vi "Parse State Queue++.vi"(0 "State Queue":string, 1 "Name (\"\" to Use UUID)":string, 2 "Response Arguments":string, 7 "Previous Error":errorcluster, 9 "Dequeue (1 ms)":i32=1, 11 "Response Timeout (-2 Use Global Settings)":i32=-2, 12 "Allowed Messages (Empty for All)":string[](array[string])) -> (3 "Name Used":string, 4 "Remaining States":string, 6 "Current State":string, 8 "Arguments":string, 10 "Additional Information":T1, 15 "Source CSM":string)   [LabVIEW 2017, in "Communicable State Machine.lvlib"]
doc: "Parses the CSM state queue and returns the next current state to execute, along with arguments and other information.\n\n\n> [!NOTE] <b>CSM Inter-module Communication Types</b>\n>\n> Communication between CSM modules is divided into two categories: Messages and Broadcasts.\n> - <b>Messages</b>: 1:1 communication between modules. Based on the message handling method, it can be further divided into Synchronous Call (`-@`), Asynchronous Call (`->`), and Asynchronous Call without Reply (`->|`).\n> - <b>Broadcasts</b>: 1:N communication between modules. The broadcasting module pushes the broadcast to all modules registered to that broadcast. Based on the broadcast processing priority, it can be further divided into Status Broadcast and Interrupt Broadcast.\n\n\n-- <b>Controls</b> --\n- <b>Response Arguments</b>: Response arguments from the previous state. Connect this input to the CSM shift register to pass return values from external calls.\n- <b>Name (\"\" to use UUID)</b>: CSM module name. Refer to <b>CSM Naming Rules</b> for module naming rules.\n- <b>State Queue</b>: The entire state queue is connected to this input. This must be wired from a CSM shift register.\n- <b>Previous Error</b>: Error cluster from the CSM. If an error occurs and is passed to this input, the <b>Current State</b> output returns the `Error Handler` state.\n- <b>Dequeue (1 ms)</b>: Timeout setting for checking the CSM message queue. The default is 1 ms. The default is not set to 0 to avoid generating massive amounts of empty messages in certain error situations.\n- <b>Response Timeout (-2 Use Global Settings)</b>: Timeout for synchronous calls. The default is -2, which uses the global setting. You can set the global timeout using the CSM - Set TMO of Sync-Reply VI.\n- <b>Allowed Messages (Empty for All)</b>: A list of allowed message names. An empty list indicates that all messages are allowed.\n\n-- <b>Indicators</b> --\n- <b>Name Used</b>: Actual name assigned to the CSM module.\n- <b>Remaining States</b>: All concatenated states and arguments.\n- <b>Current State</b>: The next current state to execute.\n- <b>Arguments</b>: Returns any arguments that might be used in the current state string. These arguments are located after the `>>` characters.\n - Argument variables must not contain any non-printable characters, such as line feeds or carriage returns.\n- <b>Additional Information</b>: Supplemental information. For states triggered by a broadcast, this information contains the name and arguments of the broadcast.\n- <b>Source CSM</b>: If <b>Current State</b> is sent externally, this is the name of the source CSM module."
uses:
  Communicable State Machine.lvlib
  _Support/Typedef/_CSM_Response Source Message.ctl
  _Support/Typedef/_CSM_MSG_TYPE.ctl
  AdvanceAPI/CSM - Message Type.ctl
  _Support/FGV-BroadcastRegistry/Operation-BroadcastRegistry.ctl
  _Support/Typedef/_CSM_GlobalLog_MSG.ctl
  _Support/Typedef/_CSM_GlobalLog_MSG_TYPE.ctl
  _Support/Typedef/_CSM Status Change Event Data.ctl
  _Support/CSMQ/_CSMObj-Message Check.vi
  _Support/CSMQ/_CSMObj-Enqueue Cross-Module Message.vi
  _Support/CSMQ/_CSMOFGV Get.vi
  _Support/GlobalEvent/GEvt-Generate with Rule Check.vi
  AdvanceAPI/CSM - Make String Arguments Safe.vi
  _Support/Common/Hex Str to U8 Data.vi
  AdvanceAPI/CSM - Revert Arguments-Safe String.vi
  _Support/Common/U8 Data to Hex Str.vi
  _Support/Priority Queue/Dequeue Element.vi
  _Support/GlobalEvent/GEvt-Convert Filter Rules - v1.0.vi
  _Support/ChangeFlag/FlagInstance-GEvt Filter.vi
  _Support/ChangeFlag/FlagInstance-GEvt Refs.vi
  _Shared/CSM - System States.vi
  _Support/Priority Queue/Enqueue Element.vi
  AdvanceAPI/CSM - Keywords.vi
  _Support/ChangeFlag/ChangeFlag-Read.vi
  _Support/GlobalEvent/LogFilter/LogFilter - Check.vi
  AdvanceAPI/CSM - Module Status.vi
  AdvanceAPI/CSM - Resolve Node Module.vi
  _Support/CSMQ/_CSMOFGV(lvlibp).vi
  _Shared/Trim Single-line Text.vi
  _Polymophic/Build Synchronous Message with Arguments.vi
  _Support/CSMKVMap/CSMKVMap-Read.vi
  _Support/Error/CSM Not Allowed Message.vi
  _Support/FGV-BroadcastRegistry/FGV-BroadcastRegistry(lvlibp).vi
  _Support/CSMQ/_CSMObj-Add Internal Registry Rule.vi
  _Support/Message/Parse Unregister Message.vi
  _Support/Message/Parse Register Message.vi
  _Shared/Concatenate State with Arguments.vi
  _Support/Error/CSM Missing Return State Error.vi
  Utility/Build Internal State String.vi
  _Shared/Concatenate PostPostMsg Message.vi
  Utility/_openG/1D Array to String_csm.vi
  _Support/GlobalEvent/LogFilter/SettingVIs/Set CSM StateType Filter.vi
  _Support/GlobalEvent/LogFilter/SettingVIs/Set Global StateType Filter.vi
  _Support/GlobalEvent/LogFilter/SettingVIs/Set CSM State Filter.vi
  _Support/GlobalEvent/LogFilter/SettingVIs/Set CSM LogType Filter.vi
  _Support/GlobalEvent/LogFilter/SettingVIs/Set Global State Filter.vi
  _Support/GlobalEvent/LogFilter/SettingVIs/Set Global LogType Filter.vi
  _Support/GlobalEvent/LogFilter/SettingVIs/Set Global CSM Filter.vi
  _Support/GlobalEvent/FGV-GEvt Filter Rules(lvlibp).vi
  _Support/ChangeFlag/ChangeFlagDB.vi
  _Support/GlobalEvent/GEvt-Valid Subscribers.vi
  _Support/GlobalEvent/FGV-GlobalEventQueues(lvlibp).vi
  _Support/GlobalEvent/FGV-GlobalEventRef(lvlibp).vi
  _Support/GlobalEvent/LogFilter/LogFilter.lvclass
  _Shared/CSM Shared.lvlib
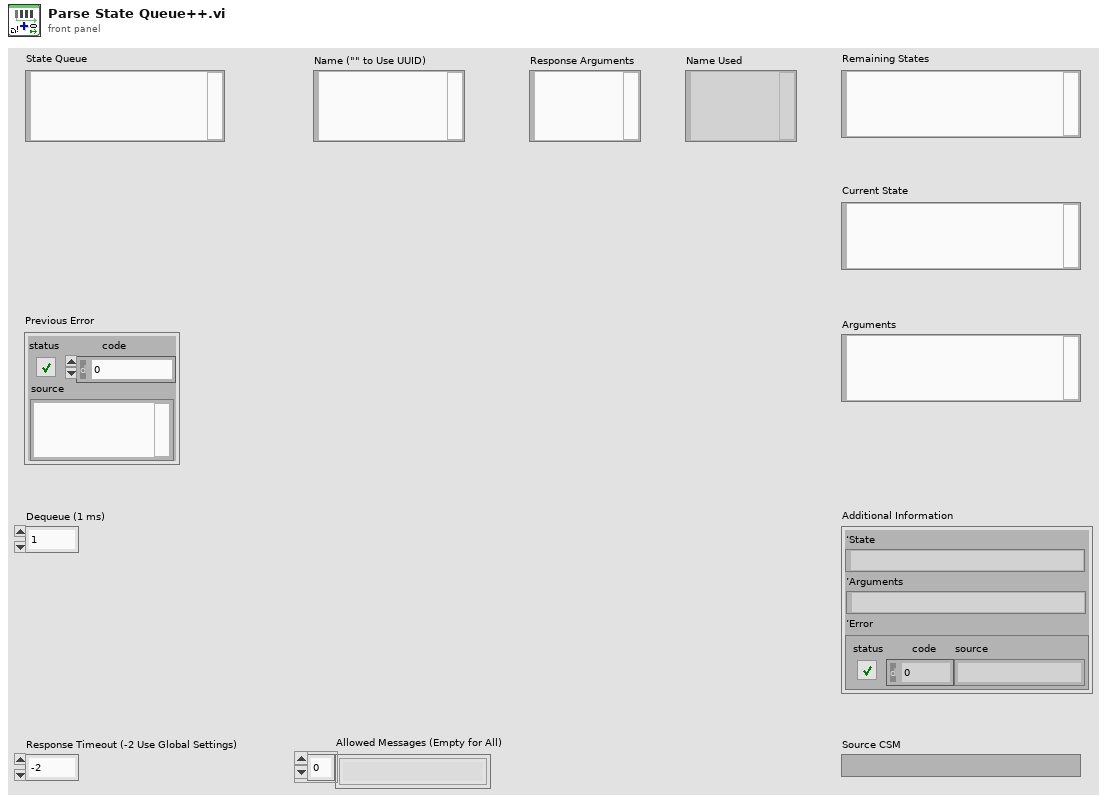
[diagram p1: front panel]
types:
  T1 = typedef "Communicable State Machine.lvlib/_CSM_Response Source Message.ctl" = cluster{"‘State":string, "’Arguments":string, "’Error":errorcluster}
  T2 = typedef "Communicable State Machine.lvlib/GEvt-Refs.ctl" = cluster{"Event":refnum<user-event>, "Queues":refnum<queue>[], "Valid":bool}
  T3 = typedef "Communicable State Machine.lvlib/_CSMObj.ctl" = cluster{"info":T4, "Refs":T6}
  T4 = typedef "Communicable State Machine.lvlib/_CSMObj-Info.ctl" = cluster{"Module Name":string, "Requested Name":string, "Group Name":string, "Mode":T5, "Allowed Messages":string[]}
  T5 = typedef "Communicable State Machine.lvlib/_CSM_MODE.ctl" = enum16{"Not Exist", "Stand Alone", "CSM", "Worker", "Worker Agent", "Chain Node", "Chain"}
  T6 = typedef "Communicable State Machine.lvlib/_CSMObj-Refs.ctl" = cluster{"WatchDogQ":refnum<queue>, "CSMDataDVR":refnum<data-value>, "Queue":T7, "GroupDataDVR":refnum<data-value>, "TagMap":refnum<data-value>, "ExitEvent":refnum<user-event>, "NewStateEvent":refnum<user-event>, "StatusEvent":refnum<user-event>, "InterruptEvent":refnum<user-event>}
  T7 = typedef "Communicable State Machine.lvlib/Priority Queue.ctl" = cluster{"HPriorityQ":refnum<queue>, "LowPriorityQ":refnum<queue>}
  T8 = typedef "Communicable State Machine.lvlib/CSM - Message Type.ctl" = enum16{"Async", "Async without Reply", "Sync"}
  T9 = typedef "Communicable State Machine.lvlib/_CSM_MSG_TYPE.ctl" = enum16{"Sync Message(-@)", "Async Message(->)", "Async without Response(->|)", "Async Response", "Broadcast(-><all>)", "Broadcast(-><status>)", "Broadcast(-><interrupt>)", "Append to JKISM States", "Append to JKISM States(High Priority)", "Broadcast(-><state>)", "<None>"}
  T10 = typedef "Communicable State Machine.lvlib/Operation-BroadcastRegistry.ctl" = enum16{"Delete Source Module", "Delete Target Module", "Remove Module", "Register", "Unregister", "Check", "List Status", "List Entries", "List Status Of Source", "Drop", "Register As Status", "Register As Interrupt"}
  T11 = typedef "Communicable State Machine.lvlib/_CSM_GlobalLog_MSG_TYPE.ctl" = enum16{"User Log", "State Change", "Status", "Interrupt", "Register", "Unregister", "Error Log", "Module Created", "Module Destroyed", "Async Message", "No-Rep Async Message", "Sync Message"}
  T12 = typedef "Communicable State Machine.lvlib/_CSM_GlobalLog_MSG.ctl" = cluster{"Name (\"\" to Use UUID)":string, "Current State":string, "Arguments":string, "Source Message":T1, "Source Module":string, "Complete(T)/Start(F)":bool, "LogType":T11, "Time Stamp":timestamp}
  T13 = typedef "Communicable State Machine.lvlib/_CSM Status Change Event Data.ctl" = cluster{"ModuleName":string, "Status":string, "Arguments":string}
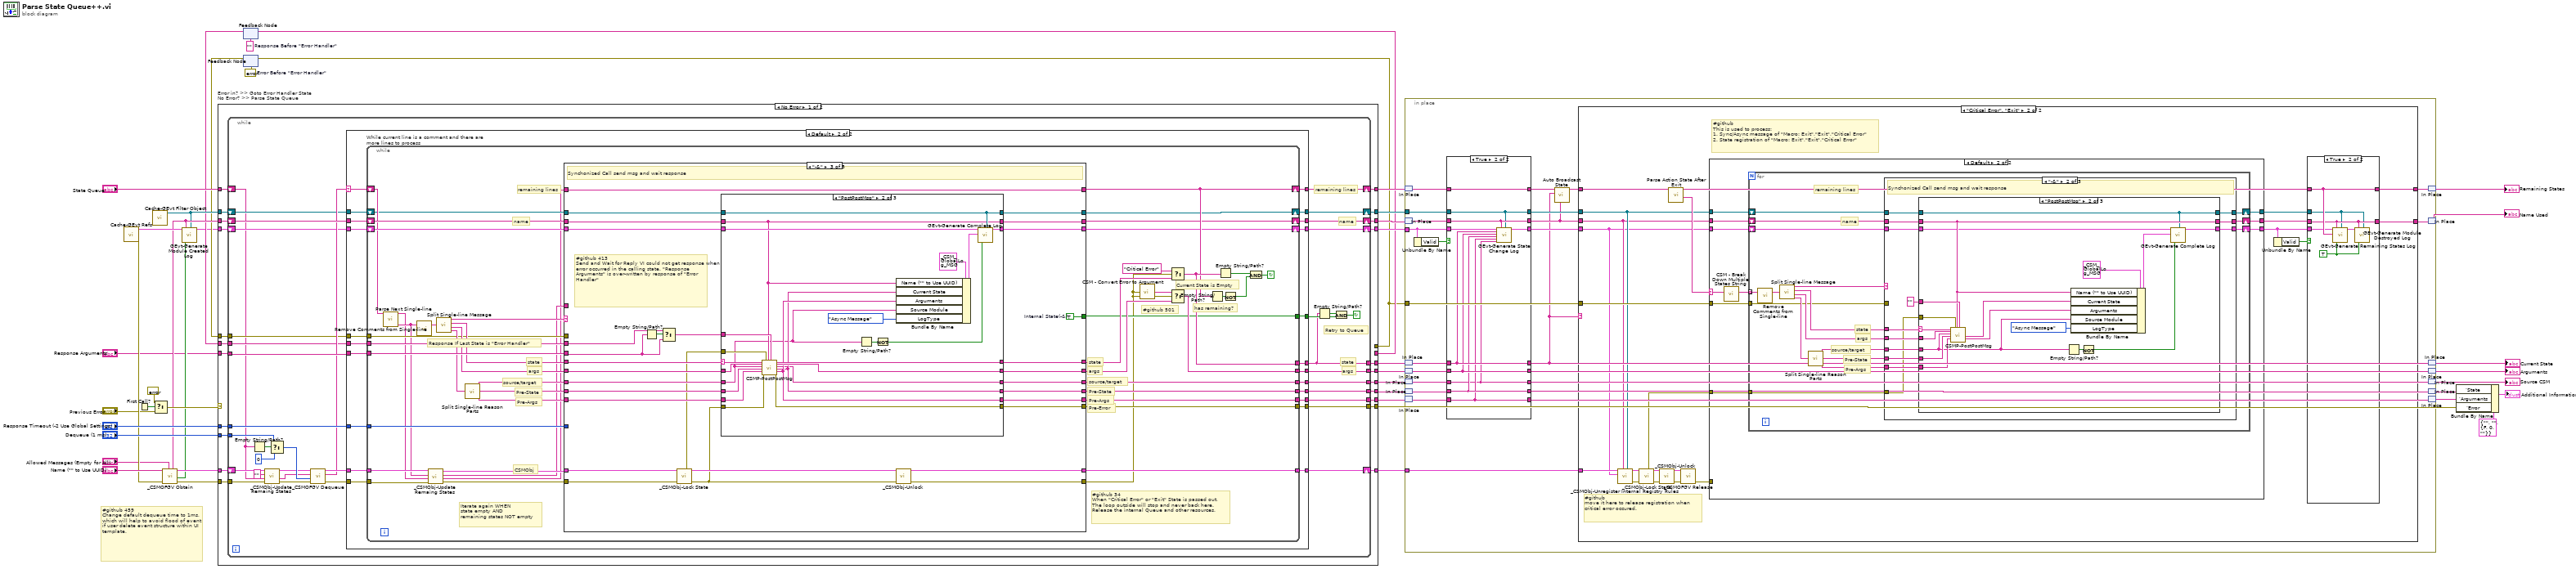
[diagram p0: block diagram]
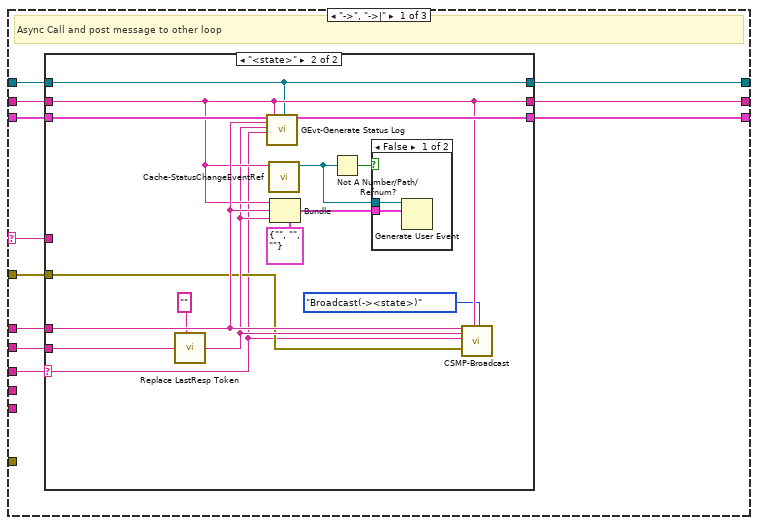
[diagram p4: hidden frame]
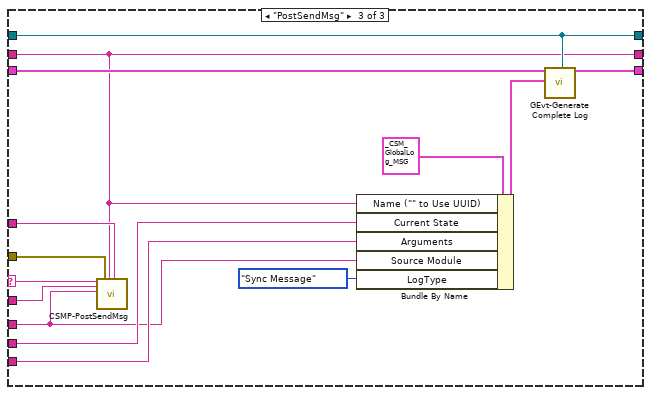
[diagram p8: hidden frame]
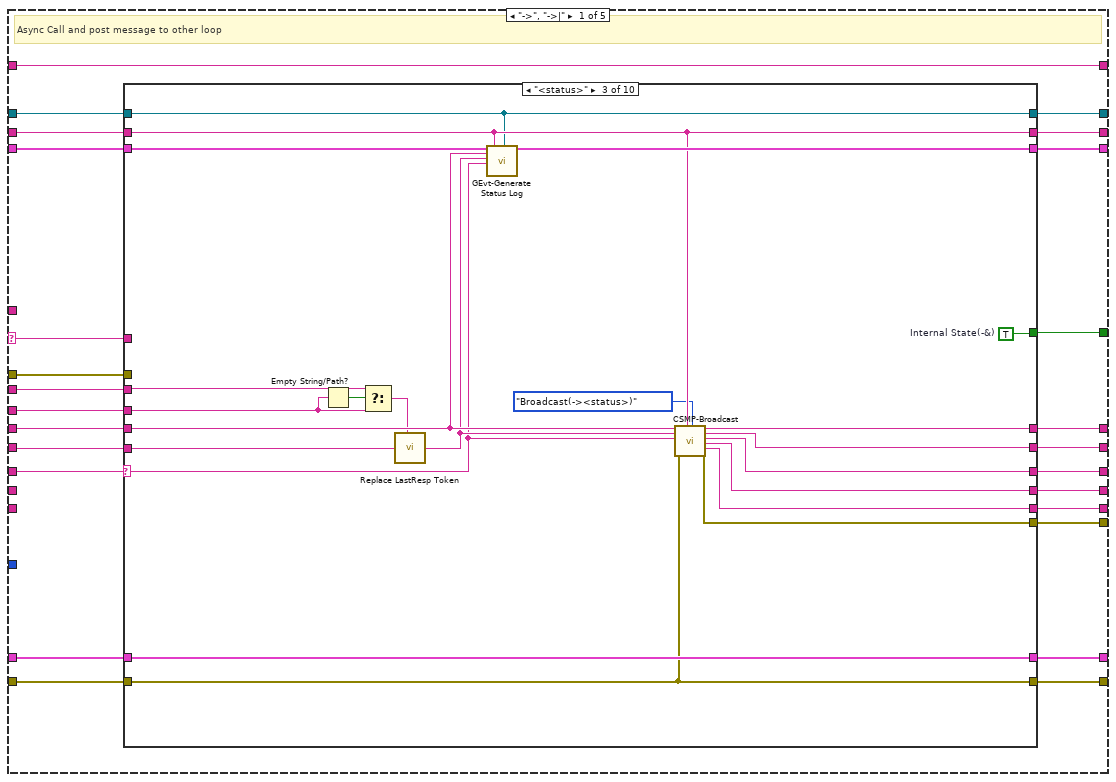
[diagram p13: hidden frame]
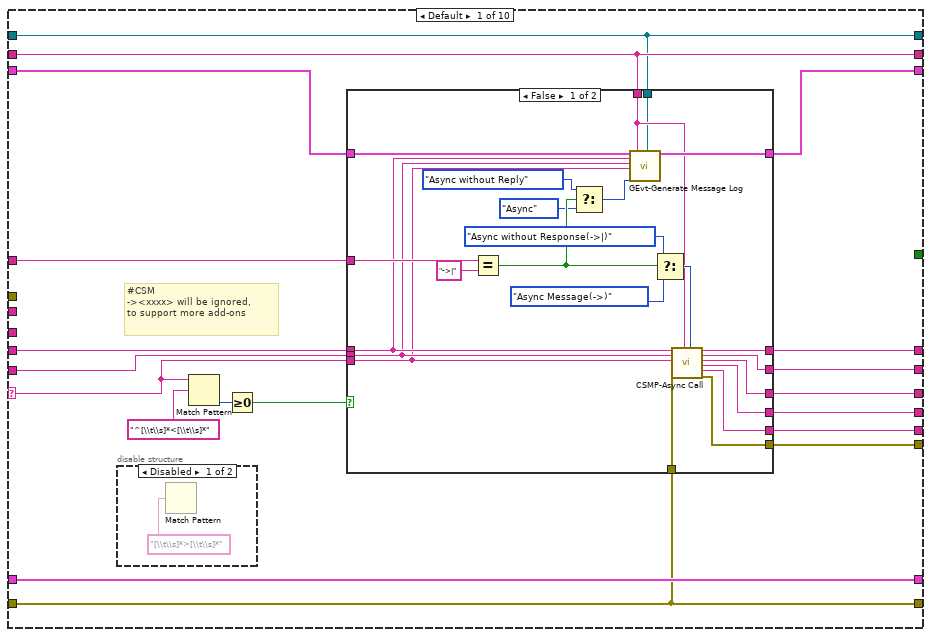
[diagram p14: hidden frame]
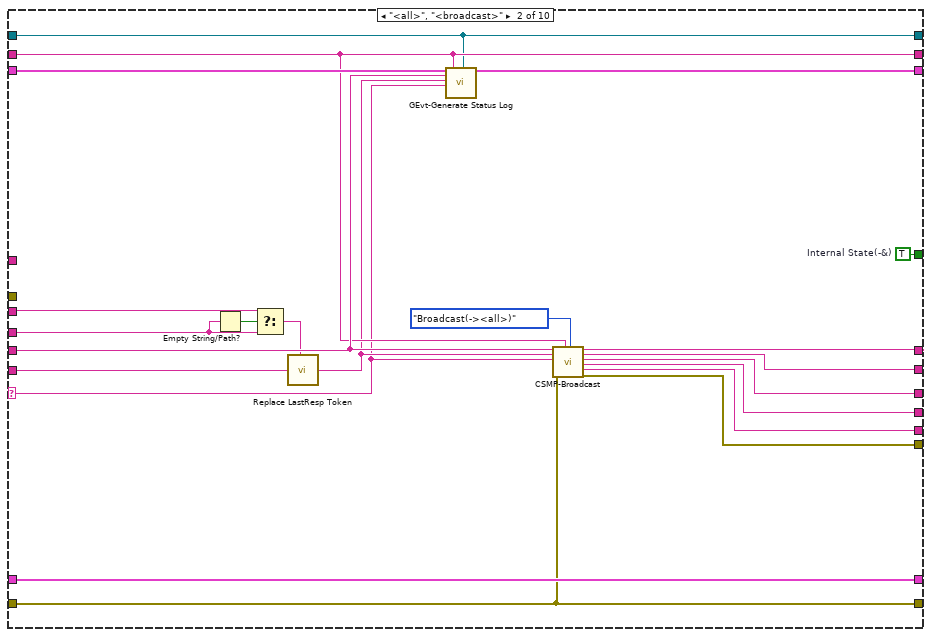
[diagram p17: hidden frame]
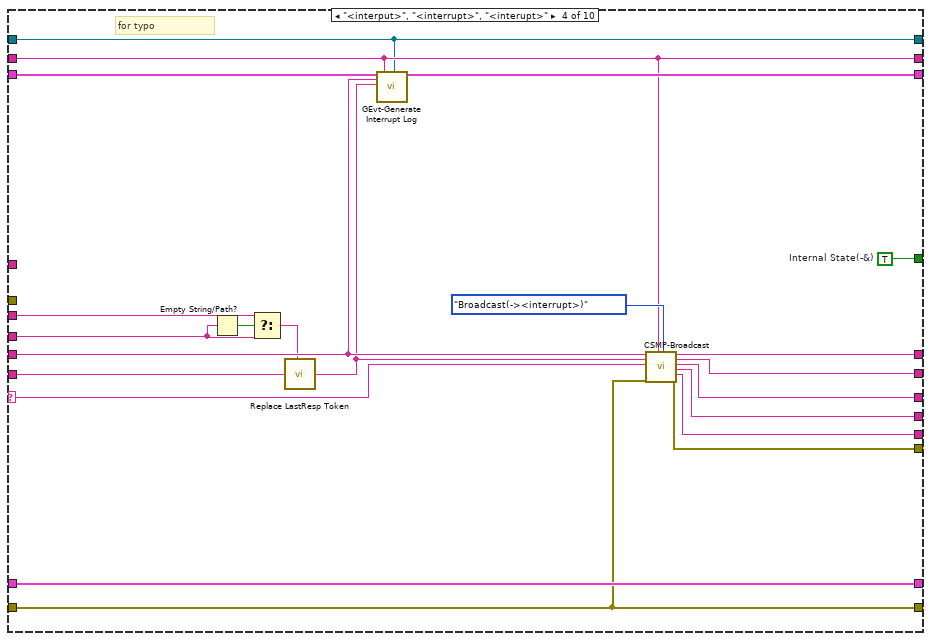
[diagram p18: hidden frame]
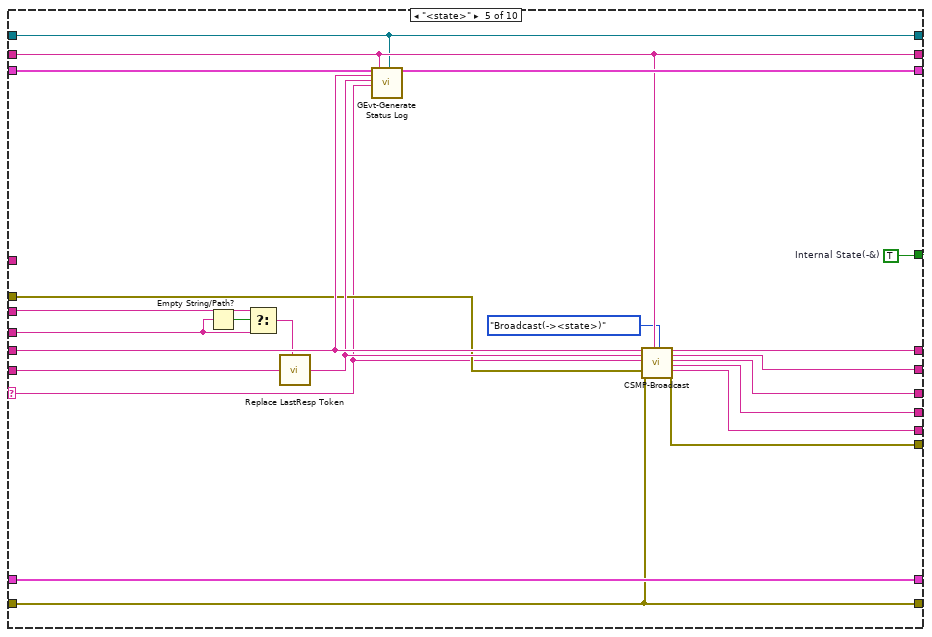
[diagram p19: hidden frame]
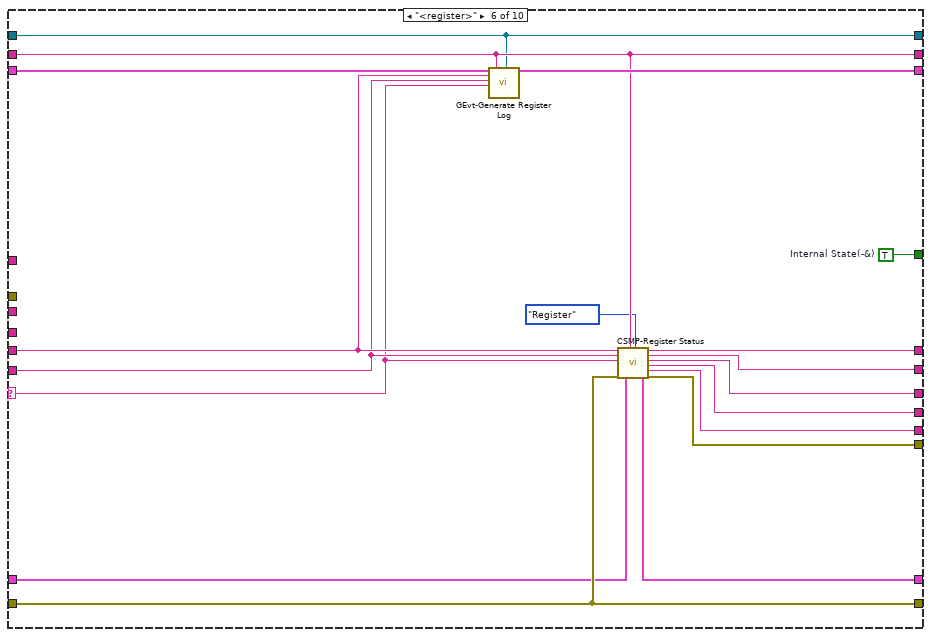
[diagram p20: hidden frame]
diagram:
  w5 = errorcluster {"status"=FALSE, "code"=0, "source"=""}  # Error Before "Error Handler"
  w8 = ""  # Response Before "Error Handler"
  # "#github 459\nChange default dequeue time to 1ms, which will help to avoid flood of event\nif user delete event structure within UI template."
  n1 = call "Cache-GEvt Refs.vi"() -> ("error out"=w28:errorcluster, "CSM Global Log Ref"=w14:T2)  [unwired: 10 in]
  n2 = First Call?() -> (First Call?: T/F=w18:bool)
  n3 = call "Cache-GEvt Filter Object.vi"() -> ("CSM:LogFilter.lvclass"=w10:refnum<class "LogFilter.lvclass">)  [unwired: 11 in]
  n4 = Select(t=errorcluster {"status"=FALSE, "code"=0, "source"=""}, s=w18, f="Previous Error") -> (s? t:f=w16:errorcluster)
  n5 = call "_CSMOFGV Obtain.vi"("Allowed Messages (Empty For All)"="Allowed Messages (Empty for All)", "Error In"=w28, "Name (\"\" to Use UUID) In"="Name (\"\" to Use UUID)") -> ("error out"=w41:errorcluster, "Create? (T)/Cached(F)"=w12:bool, "CSM-Obj"=w40:T3, "Name"=w13:string)  [unwired: 5 in]
  n6 = call "GEvt-Generate Module Created Log.vi"("CSM Global Log Event"=w14, "Name (\"\" to Use UUID)"=w13, "Created?"=w12, "CSM:LogFilter.lvclass"=w10) -> ("CSM Global Log Event Out"=w1:T2)  [unwired: 14 in, 1 out]
  n7 = feedback #1(w8) -> (w6:string)
  n8 = feedback #2(w5) -> (w4:errorcluster)
  n9 = case "Error in? >> Goto Error Handler State\nNo Error? >> Parse State Queue" shown="No Error" w16 {
    selector: w16 -> [_ w630]
    tunnel: [w64 w639] -> w31
    tunnel: [w66 "Error Handler"] -> w39
    tunnel: [w65 w635] -> w38
    tunnel: "State Queue" -> [w61 w639]
    tunnel: "Response Timeout (-2 Use Global Settings)" -> [w63 _]
    tunnel: w40 -> [w56 w634]
    tunnel: [w62 _] -> w36
    tunnel: "Dequeue (1 ms)" -> [w60 _]
    tunnel: [w59 _] -> w37
    tunnel: "Response Arguments" -> [w58 w631]
    tunnel: w41 -> [w57 w633]
    tunnel: w13 -> [w55 w637]
    tunnel: w1 -> [w54 w636]
    tunnel: [w53 w637] -> w27
    tunnel: [w52 w636] -> w26
    tunnel: [w51 _] -> w23
    tunnel: [w50 _] -> w20
    tunnel: w10 -> [w49 w632]
    tunnel: [w48 w632] -> w11
    tunnel: [_ w631] -> w7
    tunnel: w6 -> [w47 _]
    tunnel: [_ w630] -> w3
    tunnel: w4 -> [w46 _]
    tunnel: [w45 w629] -> w2
    frame No Error {
      n10 = while {
        tunnel: [w101] -> w65
        tunnel: w63 -> [w99]
        tunnel: [w98] -> w62
        tunnel: w60 -> [w95]
        tunnel: w57 -> [w73]
        shift-right: [w100] -> w64
        shift-left: w61 -> [w69]
        tunnel: w58 -> [w91]
        tunnel: [w85] -> w66
        tunnel: [w92] -> w59
        shift-right: [w82] -> w53
        shift-left: w55 -> [w90]
        shift-right: [w81] -> w52
        shift-left: w54 -> [w83]
        tunnel: [w80] -> w51
        tunnel: [w79] -> w50
        shift-right: [w77] -> w48
        shift-left: w49 -> [w78]
        tunnel: w47 -> [w76]
        tunnel: w46 -> [w75]
        shift-right: [w74] -> w45
        shift-left: w56 -> [w72]
        stop <- w87 continue-if-true
        # "args"
        # "state"
        # "name"
        # "remaining lines"
        # "Retry to Queue"
        n11 = Empty String/Path?(string/path=w69) -> (empty?=w96:bool)
        n12 = call "_CSMObj-Update Remaing States.vi"("Error In"=w73, "Remaing JKISM Queue"=w69, "Current State"="", "CSMQ In"=w72) -> ("error out"=w70:errorcluster, "Remaing JKISM Queue(dup)"=w68:string, "CSMQ Out"=w71:T3)  [unwired: 4 in, 1 out]
        n13 = Select(t=w95, s=w96, f=0) -> (s? t:f=w93:i32)
        n14 = call "_CSMOFGV Dequeue.vi"("Error In"=w70, "Dequeue Timeout (0ms)"=w93, "State (S) In (\"\")"=w68, "CSMQ In"=w71) -> ("error out"=w88:errorcluster, "States Out"=w89:string, "CSMQ Out"=w97:T3)  [unwired: 5 in]
        n15 = case shown="Default" w89 {
          selector: w89 -> [_ w121]
          tunnel: [_ w127] -> w85
          tunnel: [_ w126] -> w101
          tunnel: [_ w125] -> w100
          tunnel: w99 -> [_ w124]
          tunnel: [_ w123] -> w98
          tunnel: w90 -> [w105 w122]
          tunnel: w97 -> [w102 w120]
          tunnel: w88 -> [_ w119]
          tunnel: [_ w118] -> w92
          tunnel: w91 -> [_ w117]
          tunnel: [_ w116] -> w86
          tunnel: w83 -> [w104 w115]
          tunnel: [w105 w114] -> w82
          tunnel: [w104 w113] -> w81
          tunnel: [_ w112] -> w80
          tunnel: [_ w111] -> w79
          tunnel: w78 -> [w103 w110]
          tunnel: [w103 w109] -> w77
          tunnel: w76 -> [_ w108]
          tunnel: w75 -> [_ w107]
          tunnel: [w102 w106] -> w74
          frame "" {
            # "Dispatch Mode\n1. Error will Occurred\n2. Add Macro: Exit\n3. The Queue will regenerated\n4. But it will go Through Macro: Exit\n5. After Exit(queue released), then another Worker will be triggered."
            # "Do Nothing if Empty String"
            # "<< Wiring into the Case Selector is much more performant than using \"Empty String/Path?\" primitive"
          }
          frame Default {
            n16 = while "While current line is a comment and there are more lines to process" {
              tunnel: [w162] -> w127
              tunnel: [w164] -> w126
              shift-right: [w158] -> w125
              shift-left: w121 -> [w150]
              tunnel: w124 -> [w169]
              tunnel: [w163] -> w123
              tunnel: w120 -> [w134]
              tunnel: w119 -> [w135]
              tunnel: [w168] -> w118
              tunnel: w117 -> [w167]
              tunnel: [w160] -> w116
              shift-right: [w141] -> w114
              shift-left: w122 -> [w157]
              shift-right: [w139] -> w113
              shift-left: w115 -> [w156]
              tunnel: [w155] -> w112
              tunnel: [w145] -> w111
              shift-right: [w140] -> w109
              shift-left: w110 -> [w142]
              tunnel: w108 -> [w144]
              tunnel: w107 -> [w143]
              tunnel: [w138] -> w106
              stop <- w159 continue-if-true
              # "#github 501"
              # "Response If Last State is \"Error Handler\""
              # "source/target"
              # "Pre-Error"
              # "args"
              # "state"
              # "Pre-Args"
              # "Pre-State"
              # "source/target"
              # "Pre-Args"
              # "Pre-State"
              # "CSMObj"
              # "#github 34\nWhen \"Critical Error\" or \"Exit\" State is passed out,\nThe loop outside will stop and never back here.\nRelease the internal Queue and other resources."
              # "name"
              # "remaining lines"
              # "Iterate again WHEN\nstate empty AND\nremaining states NOT empty"
              # "args"
              # "state"
              # "Current State is Empty"
              # "has remaining?"
              n17 = call "Parse Next Single-line.vi"("States Queue"=w150) -> ("Next Single-line State"=w131:string, "Remaining States Queue"=w130:string)  [unwired: 9 in]
              n18 = call "Remove Comments from Single-line.vi"("single-line text"=w131) -> ("single-line text without comments"=w154:string)  [unwired: 2 in]
              n19 = call "_CSMObj-Update Remaing States.vi"("Error In"=w135, "Remaing JKISM Queue"=w130, "Current State"=w131, "CSMQ In"=w134) -> ("error out"=w132:errorcluster, "Remaing JKISM Queue(dup)"=w128:string, "Current State(dup)"=w129:string, "CSMQ Out"=w133:T3)  [unwired: 4 in]
              n20 = call "Split Single-line Message.vi"("single-line text"=w154) -> ("operator"=w151:string, "state"=w152:string, "args"=w153:string, "source/target"=w149:string)  [unwired: 6 in]
              n21 = call "Split Single-line Reason Parts.vi"("Single-line -& Reason"=w149) -> ("CSM Name"=w148:string, "`State"=w147:string, "`Arguments"=w146:string)  [unwired: 12 in]
              n22 = case shown="\"-&\"" w151 {
                selector: w151 -> [w186 _ _ _ _]
                tunnel: w152 -> [w194 w423 w463 w537 w628]
                tunnel: w153 -> [w193 w422 w465 w536 w627]
                tunnel: [w197 w435 w467 w535 w628] -> w166
                tunnel: [w196 w434 w466 w534 w627] -> w165
                tunnel: w157 -> [w192 w425 w457 w529 w621]
                tunnel: w148 -> [w195 w421 w456 w532 w624]
                tunnel: w169 -> [_ w428 _ _ _]
                tunnel: w133 -> [w184 w437 w451 w543 w625]
                tunnel: w128 -> [w187 w436 w459 w539 w623]
                tunnel: [w191 w432 w462 w531 _] -> w168
                tunnel: w167 -> [w189 _ w445 _ _]
                tunnel: w132 -> [w190 w429 w450 w542 w626]
                tunnel: [w177 w429 w464 w541 w626] -> w137
                tunnel: [w179 w433 w453 w533 w624] -> w163
                tunnel: [w185 w437 w461 w540 w625] -> w138
                tunnel: [w188 _ w460 w527 _] -> w160
                tunnel: [w187 w436 w459 w538 w623] -> w158
                tunnel: w156 -> [w183 w427 w438 w528 w622]
                tunnel: [w182 w426 w439 w528 w622] -> w139
                tunnel: [w180 w431 w458 w522 _] -> w155
                tunnel: [w181 w425 w442 w529 w621] -> w141
                tunnel: w147 -> [_ _ w455 w530 _]
                tunnel: w146 -> [_ _ w454 w523 _]
                tunnel: [w178 w430 w452 w521 _] -> w145
                tunnel: w142 -> [w176 w424 w440 w520 w620]
                tunnel: w129 -> [_ _ _ w526 _]
                tunnel: w144 -> [w175 _ w444 _ _]
                tunnel: w143 -> [w174 _ _ _ _]
                tunnel: [w173 w424 w441 w520 w620] -> w140
                frame "->", "->|" {
                  # "Async Call and post message to other loop"
                  n23 = case shown="\"<status>\"" w195 {
                    selector: w195 -> [w203 w246 w268 w301 w312 w334 w352 w370 w402 _]
                    tunnel: [w211 w252 w281 w300 w328 w349 w367 w385 w401 _] -> w197
                    tunnel: [w210 w253 w278 w299 w325 w348 w366 w384 w400 _] -> w196
                    tunnel: w194 -> [w216 w262 w282 w303 w329 w338 w356 w374 w390 w406]
                    tunnel: w193 -> [w212 w261 w279 w302 w326 w337 w355 w373 w389 _]
                    tunnel: w192 -> [w213 w260 w280 w305 w327 w339 w357 w375 w391 w412]
                    tunnel: [w209 w255 w276 w297 w323 w346 w364 w382 w398 _] -> w191
                    tunnel: w190 -> [w205 w258 w284 w304 w314 w350 w368 w386 w403 w408]
                    tunnel: w189 -> [_ w248 w271 w291 w318 _ _ _ _ _]
                    tunnel: [_ w266 w288 w310 w333 w351 w369 w387 w404 TRUE ("Internal State(-&)")] -> w188
                    tunnel: w186 -> [w215 _ _ _ _ _ _ _ _ _]
                    tunnel: [w214 w265 w287 w309 w315 w342 w360 w378 w394 w410] -> w185
                    tunnel: w184 -> [w214 w265 w287 w309 w315 w343 w361 w379 w395 w409]
                    tunnel: [w199 w264 w285 w307 w331 w340 w358 w376 w392 w413] -> w182
                    tunnel: w183 -> [w200 w263 w286 w308 w332 w341 w359 w377 w393 w413]
                    tunnel: [w213 w260 w280 w305 w327 w339 w357 w375 w391 w412] -> w181
                    tunnel: [w208 w256 w275 w296 w322 w345 w363 w381 w397 _] -> w180
                    tunnel: [w207 w254 w277 w298 w324 w347 w365 w383 w399 _] -> w179
                    tunnel: [w206 w257 w283 w295 w330 w344 w362 w380 w396 _] -> w178
                    tunnel: [w205 w258 w284 w304 w314 w350 w368 w386 w403 w407] -> w177
                    tunnel: w176 -> [w198 w245 w267 w289 w311 w336 w354 w372 w388 w405]
                    tunnel: w175 -> [_ w249 w270 w292 w317 _ _ _ _ _]
                    tunnel: w174 -> [_ _ _ _ w313 _ _ _ _ _]
                    tunnel: [w198 w245 w267 w289 w311 w336 w354 w372 w388 w405] -> w173
                    frame Default {
                      # "#CSM\n-><xxxx> will be ignored,\nto support more add-ons"
                      n24 = disable-structure shown="Disabled" {
                        frame Disabled {
                          n25 = Match Pattern(regular expression="[\\t\\s]*>[\\t\\s]*") -> ()  [unwired: 2 in, 4 out]
                        }
                        frame Enabled {
                        }
                      }
                      n26 = Match Pattern(string=w203, regular expression="^[\\t\\s]*<[\\t\\s]*") -> (offset past match=w202:i32)  [unwired: 1 in, 3 out]
                      n27 = Greater Or Equal To 0?(x=w202) -> (x >= 0?=w201:bool)
                      n28 = case shown="False" w201 {
                        tunnel: w216 -> [w224 w244]
                        tunnel: w215 -> [w240 _]
                        tunnel: w213 -> [w226 _]
                        tunnel: w212 -> [w223 w243]
                        tunnel: [w236 w244] -> w211
                        tunnel: [w235 w243] -> w210
                        tunnel: [w234 _] -> w209
                        tunnel: [w233 _] -> w208
                        tunnel: [w232 w242] -> w207
                        tunnel: [w231 _] -> w206
                        tunnel: w205 -> [w229 _]
                        tunnel: w203 -> [w222 w242]
                        tunnel: w200 -> [w228 w241]
                        tunnel: [w227 w241] -> w199
                        tunnel: w198 -> [w225 _]
                        frame False {
                          n29 = Equal?(x=w240, y="->|") -> (x = y?=w220:bool)
                          n30 = Select(t=CSM_-_Message_Type."Async without Reply" ("Type"), s=w220, f=CSM_-_Message_Type."Async" ("Type")) -> (s? t:f=w218:T8)
                          n31 = call "GEvt-Generate Message Log.vi"("CSM Global Log Event"=w228, "Current State"=w224, "Arguments"=w223, "Source Module"=w222, "Type"=w218, "Name (\"\" to Use UUID)"=w226, "CSM:LogFilter.lvclass"=w225) -> ("CSM Global Log Event Out"=w227:T2)  [unwired: 11 in, 1 out]
                          n32 = Select(t=_CSM_MSG_TYPE."Async without Response(->|)" ("Msg Type"), s=w220, f=_CSM_MSG_TYPE."Async Message(->)" ("Msg Type")) -> (s? t:f=w230:T9)
                          n33 = call "CSMP-Async Call.vi"("State"=w224, "Args"=w223, "Source/target"=w222, "Error In"=w229, "Module Name"=w226, "Msg Type"=w230) -> ("State Out"=w236:string, "Args Out"=w235:string, "Source/target Out"=w232:string, "Pre-State Out"=w234:string, "Pre-Args Out"=w233:string, "Error"=w231:errorcluster)  [unwired: 8 in]
                        }
                        frame True {
                        }
                      }
                    }
                    frame "<all>", "<broadcast>" {
                      w266 = TRUE  # Internal State(-&)
                      n34 = Empty String/Path?(string/path=w248) -> (empty?=w250:bool)
                      n35 = Select(t=w249, s=w250, f=w248) -> (s? t:f=w247:string)
                      n36 = call "Replace LastResp Token.vi"("LastResp"=w247, "Argument"=w261) -> ("Argument Out"=w251:string)  [unwired: 5 in]
                      n37 = call "GEvt-Generate Status Log.vi"("CSM Global Log Event"=w263, "Current State"=w262, "Arguments"=w251, "Source Module"=w246, "Name (\"\" to Use UUID)"=w260, "CSM:LogFilter.lvclass"=w245) -> ("CSM Global Log Event Out"=w264:T2)  [unwired: 12 in, 1 out]
                      n38 = call "CSMP-Broadcast.vi"("State"=w262, "Args"=w251, "Source/target"=w246, "Error In"=w258, "Module Name"=w260, "Msg Type"=_CSM_MSG_TYPE."Broadcast(-><all>)") -> ("State Out"=w252:string, "Args Out"=w253:string, "Source/target Out"=w254:string, "Pre-State Out"=w255:string, "Pre-Args Out"=w256:string, "Error"=w257:errorcluster)  [unwired: 8 in]
                    }
                    frame "<status>" {
                      w288 = TRUE  # Internal State(-&)
                      n39 = Empty String/Path?(string/path=w271) -> (empty?=w272:bool)
                      n40 = Select(t=w270, s=w272, f=w271) -> (s? t:f=w269:string)
                      n41 = call "Replace LastResp Token.vi"("LastResp"=w269, "Argument"=w279) -> ("Argument Out"=w273:string)  [unwired: 5 in]
                      n42 = call "GEvt-Generate Status Log.vi"("CSM Global Log Event"=w286, "Current State"=w282, "Arguments"=w273, "Source Module"=w268, "Name (\"\" to Use UUID)"=w280, "CSM:LogFilter.lvclass"=w267) -> ("CSM Global Log Event Out"=w285:T2)  [unwired: 12 in, 1 out]
                      n43 = call "CSMP-Broadcast.vi"("State"=w282, "Args"=w273, "Source/target"=w268, "Error In"=w284, "Module Name"=w280, "Msg Type"=_CSM_MSG_TYPE."Broadcast(-><status>)") -> ("State Out"=w281:string, "Args Out"=w278:string, "Source/target Out"=w277:string, "Pre-State Out"=w276:string, "Pre-Args Out"=w275:string, "Error"=w283:errorcluster)  [unwired: 8 in]
                    }
                    frame "<interput>", "<interrupt>", "<interupt>" {
                      w310 = TRUE  # Internal State(-&)
                      # "for typo"
                      n44 = Empty String/Path?(string/path=w291) -> (empty?=w293:bool)
                      n45 = Select(t=w292, s=w293, f=w291) -> (s? t:f=w290:string)
                      n46 = call "Replace LastResp Token.vi"("LastResp"=w290, "Argument"=w302) -> ("Argument Out"=w294:string)  [unwired: 5 in]
                      n47 = call "GEvt-Generate Interrupt Log.vi"("CSM Global Log Event"=w308, "Current State"=w303, "Arguments"=w294, "Name (\"\" to Use UUID)"=w305, "CSM:LogFilter.lvclass"=w289) -> ("CSM Global Log Event Out"=w307:T2)  [unwired: 13 in, 1 out]
                      n48 = call "CSMP-Broadcast.vi"("State"=w303, "Args"=w294, "Source/target"=w301, "Error In"=w304, "Module Name"=w305, "Msg Type"=_CSM_MSG_TYPE."Broadcast(-><interrupt>)") -> ("State Out"=w300:string, "Args Out"=w299:string, "Source/target Out"=w298:string, "Pre-State Out"=w297:string, "Pre-Args Out"=w296:string, "Error"=w295:errorcluster)  [unwired: 8 in]
                    }
                    frame "<state>" {
                      w333 = TRUE  # Internal State(-&)
                      n49 = Empty String/Path?(string/path=w318) -> (empty?=w319:bool)
                      n50 = Select(t=w317, s=w319, f=w318) -> (s? t:f=w316:string)
                      n51 = call "Replace LastResp Token.vi"("LastResp"=w316, "Argument"=w326) -> ("Argument Out"=w320:string)  [unwired: 5 in]
                      n52 = call "GEvt-Generate Status Log.vi"("CSM Global Log Event"=w332, "Current State"=w329, "Arguments"=w320, "Source Module"=w312, "Name (\"\" to Use UUID)"=w327, "CSM:LogFilter.lvclass"=w311) -> ("CSM Global Log Event Out"=w331:T2)  [unwired: 12 in, 1 out]
                      n53 = call "CSMP-Broadcast.vi"("State"=w329, "Args"=w320, "Source/target"=w312, "Response For Message.’Error"=w313, "Error In"=w314, "Module Name"=w327, "Msg Type"=_CSM_MSG_TYPE."Broadcast(-><state>)") -> ("State Out"=w328:string, "Args Out"=w325:string, "Source/target Out"=w324:string, "Pre-State Out"=w323:string, "Pre-Args Out"=w322:string, "Error"=w330:errorcluster)  [unwired: 7 in]
                    }
                    frame "<register>" {
                      w351 = TRUE  # Internal State(-&)
                      n54 = call "GEvt-Generate Register Log.vi"("CSM Global Log Event"=w341, "Current State"=w338, "Arguments"=w337, "Source Module"=w334, "Name (\"\" to Use UUID)"=w339, "CSM:LogFilter.lvclass"=w336) -> ("CSM Global Log Event Out"=w340:T2)  [unwired: 12 in, 1 out]
                      n55 = call "CSMP-Register Status.vi"("State"=w338, "Args"=w337, "Source/target"=w334, "Error In"=w350, "CSMQ In"=w343, "Module Name"=w339, "Operation"=Operation-BroadcastRegistry."Register") -> ("CSMQ Out"=w342:T3, "State Out"=w349:string, "Args Out"=w348:string, "Source/target Out"=w347:string, "Pre-State Out"=w346:string, "Pre-Args Out"=w345:string, "Error"=w344:errorcluster)  [unwired: 6 in]
                    }
                    frame "<register as status>" {
                      w369 = TRUE  # Internal State(-&)
                      n56 = call "GEvt-Generate Register Log.vi"("CSM Global Log Event"=w359, "Current State"=w356, "Arguments"=w355, "Source Module"=w352, "Name (\"\" to Use UUID)"=w357, "CSM:LogFilter.lvclass"=w354) -> ("CSM Global Log Event Out"=w358:T2)  [unwired: 12 in, 1 out]
                      n57 = call "CSMP-Register Status.vi"("State"=w356, "Args"=w355, "Source/target"=w352, "Error In"=w368, "CSMQ In"=w361, "Module Name"=w357, "Operation"=Operation-BroadcastRegistry."Register As Status") -> ("CSMQ Out"=w360:T3, "State Out"=w367:string, "Args Out"=w366:string, "Source/target Out"=w365:string, "Pre-State Out"=w364:string, "Pre-Args Out"=w363:string, "Error"=w362:errorcluster)  [unwired: 6 in]
                    }
                    frame "<register as interput>", "<register as interrupt>", "<register as interupt>" {
                      w387 = TRUE  # Internal State(-&)
                      n58 = call "GEvt-Generate Register Log.vi"("CSM Global Log Event"=w377, "Current State"=w374, "Arguments"=w373, "Source Module"=w370, "Name (\"\" to Use UUID)"=w375, "CSM:LogFilter.lvclass"=w372) -> ("CSM Global Log Event Out"=w376:T2)  [unwired: 12 in, 1 out]
                      n59 = call "CSMP-Register Status.vi"("State"=w374, "Args"=w373, "Source/target"=w370, "Error In"=w386, "CSMQ In"=w379, "Module Name"=w375, "Operation"=Operation-BroadcastRegistry."Register As Interrupt") -> ("CSMQ Out"=w378:T3, "State Out"=w385:string, "Args Out"=w384:string, "Source/target Out"=w383:string, "Pre-State Out"=w382:string, "Pre-Args Out"=w381:string, "Error"=w380:errorcluster)  [unwired: 6 in]
                    }
                    frame "<unregister>" {
                      w404 = TRUE  # Internal State(-&)
                      n60 = call "GEvt-Generate Unregister Log.vi"("CSM Global Log Event"=w393, "Current State"=w390, "Arguments"=w389, "Name (\"\" to Use UUID)"=w391, "CSM:LogFilter.lvclass"=w388) -> ("CSM Global Log Event Out"=w392:T2)  [unwired: 13 in, 1 out]
                      n61 = call "CSMP-Unregister Status.vi"("State"=w390, "Args"=w389, "Source/target"=w402, "Error In"=w403, "CSMQ In"=w395, "Module Name"=w391) -> ("CSMQ Out"=w394:T3, "State Out"=w401:string, "Args Out"=w400:string, "Source/target Out"=w399:string, "Pre-State Out"=w398:string, "Pre-Args Out"=w397:string, "Error"=w396:errorcluster)  [unwired: 7 in]
                    }
                    frame "<complete>" {
                      n62 = case shown="\"Macro: Initialize\"" w406 {
                        tunnel: [w415 w416] -> w410
                        tunnel: w409 -> [w415 w417]
                        tunnel: w408 -> [w414 w419]
                        tunnel: [w414 w418] -> w407
                        frame Default {
                        }
                        frame "Macro: Initialize" {
                          n63 = call "_CSMObj-Mark as Initialized.vi"("Error In"=w419, "CSMQ In"=w417) -> ("error out"=w418:errorcluster, "CSMQ Out"=w416:T3)  [unwired: 8 in]
                        }
                      }
                    }
                  }
                }
                frame "-@" {
                  # "Synchonized Call send msg and wait response"
                  n64 = call "GEvt-Generate Message Log.vi"("CSM Global Log Event"=w427, "Current State"=w423, "Arguments"=w422, "Source Module"=w421, "Type"=CSM_-_Message_Type."Sync", "Name (\"\" to Use UUID)"=w425, "CSM:LogFilter.lvclass"=w424) -> ("CSM Global Log Event Out"=w426:T2)  [unwired: 11 in, 1 out]
                  n65 = call "CSMP-Sync Call.vi"("State"=w423, "Args"=w422, "Source/target"=w421, "Error In"=w429, "Response Timeout (-2 Using Global Settings)"=w428, "Module Name"=w425) -> ("State Out"=w435:string, "Args Out"=w434:string, "Source/target Out"=w433:string, "Pre-State Out"=w432:string, "Pre-Args Out"=w431:string, "Error"=w430:errorcluster)  [unwired: 8 in]
                }
                frame "-&" {
                  w460 = TRUE  # Internal State(-&)
                  # "#github 413\nSend and Wait for Reply VI could not get response when error occurred in the calling state. \"Response Arguments\" is over-written by response of \"Error Handler\""
                  # "Synchonized Call send msg and wait response"
                  n66 = Empty String/Path?(string/path=w445) -> (empty?=w446:bool)
                  n67 = Select(t=w444, s=w446, f=w445) -> (s? t:f=w443:string)
                  n68 = call "_CSMObj-Lock State.vi"("Error In"=w450, "CSMQ In"=w451) -> ("error out"=w448:errorcluster, "CSMQ Out"=w449:T3, "Error"=w447:errorcluster)  [unwired: 5 in, 1 out]
                  n69 = case shown="\"PostPostMsg\"" w463 {
                    selector: w463 -> [w473 w497 w519]
                    tunnel: ["Critical Error" ("before match") w492 w518] -> w467
                    tunnel: [w475 w493 w516] -> w466
                    tunnel: w456 -> [_ w478 w501]
                    tunnel: w465 -> [_ w496 w517]
                    tunnel: w443 -> [_ w498 w512]
                    tunnel: w448 -> [_ w500 w515]
                    tunnel: w457 -> [w470 w485 w505]
                    tunnel: [w472 w483 w504] -> w462
                    tunnel: w455 -> [w472 w495 w504]
                    tunnel: w454 -> [w471 w494 w503]
                    tunnel: [w471 w484 w503] -> w458
                    tunnel: [_ w499 w514] -> w452
                    tunnel: [_ w481 w502] -> w453
                    tunnel: w447 -> [_ w491 w513]
                    tunnel: [w470 w485 w505] -> w442
                    tunnel: [w469 w488 w507] -> w441
                    tunnel: w440 -> [w469 w488 w507]
                    tunnel: [w468 w489 w508] -> w439
                    tunnel: w438 -> [w468 w490 w509]
                    frame Default {
                      n70 = Concatenate Strings("Framework error, it recieved \"" ("before match"), w473, "\" which is not expected." ("before match")) -> (w475:string)
                    }
                    frame "PostPostMsg" {
                      n71 = call "CSMP-PostPostMsg.vi"("State"=w497, "Args"=w496, "Source/target"=w478, "Pre-State In"=w495, "Pre-Args In"=w494, "Error In"=w500, "Session Error"=w491, "Module Name"=w485, "Response Arguments"=w498) -> ("State Out"=w492:string, "Args Out"=w493:string, "Source/target Out"=w481:string, "Pre-State Out"=w483:string, "Pre-Args Out"=w484:string, "Error"=w499:errorcluster)  [unwired: 5 in]
                      n72 = Empty String/Path?(string/path=w478) -> (empty?=w480:bool)
                      n73 = Not(x=w480) -> (.not. x?=w479:bool)
                      n74 = Bundle By Name(cluster=T12 {"Name (\"\" to Use UUID)"="", "Current State"="", "Arguments"="", "Source Message"={"‘State"="", "’Arguments"="", "’Error"={"status"=FALSE, "code"=0, "source"=""}}, "Source Module"="", "Complete(T)/Start(F)"=FALSE, "LogType"=enum."State Change", "Time Stamp"=timestamp(0 s since 1904-01-01)} ("Event Data"), "Name (\"\" to Use UUID)"=w485, "Current State"=w483, "Arguments"=w484, "Source Module"=w478, "LogType"=_CSM_GlobalLog_MSG_TYPE."Async Message") -> (w486:T12)
                      n75 = call "GEvt-Generate Complete Log.vi"("CSM Global Log Event"=w490, "Event Data"=w486, "Enable?"=w479, "CSM:LogFilter.lvclass"=w488) -> ("CSM Global Log Event Out"=w489:T2)  [unwired: 15 in]
                    }
                    frame "PostSendMsg" {
                      n76 = call "CSMP-PostSendMsg.vi"("State"=w519, "Args"=w517, "Source/target"=w501, "Error In"=w515, "Session Error"=w513, "Module Name"=w505, "Response Arguments"=w512) -> ("State Out"=w518:string, "Args Out"=w516:string, "Source/target Out"=w502:string, "Error"=w514:errorcluster)  [unwired: 9 in]
                      n77 = Bundle By Name(cluster=T12 {"Name (\"\" to Use UUID)"="", "Current State"="", "Arguments"="", "Source Message"={"‘State"="", "’Arguments"="", "’Error"={"status"=FALSE, "code"=0, "source"=""}}, "Source Module"="", "Complete(T)/Start(F)"=FALSE, "LogType"=enum."State Change", "Time Stamp"=timestamp(0 s since 1904-01-01)} ("Event Data"), "Name (\"\" to Use UUID)"=w505, "Current State"=w504, "Arguments"=w503, "Source Module"=w501, "LogType"=_CSM_GlobalLog_MSG_TYPE."Sync Message") -> (w506:T12)
                      n78 = call "GEvt-Generate Complete Log.vi"("CSM Global Log Event"=w509, "Event Data"=w506, "CSM:LogFilter.lvclass"=w507) -> ("CSM Global Log Event Out"=w508:T2)  [unwired: 16 in]
                    }
                  }
                  n79 = call "_CSMObj-Unlock.vi"("Error In"=w448, "CSMQ In"=w449) -> ("error out"=w464:errorcluster, "CSMQ Out"=w461:T3)  [unwired: 8 in]
                }
                frame "", "<-", "@-", "|<-" {
                  # "\"<-\"  : Added by Other JKI State Loop |  \"\" : Added by Current Loop"
                  n80 = Match Pattern(string=w523, regular expression="[\\t\\s]*>>>[\\t\\s]*") -> (before substring=w522:string, after substring=w525:string)  [unwired: 1 in, 2 out]
                  n81 = call "CSM - Convert Argument to Error.vi"("Argument"=w525) -> ("Error"=w521:errorcluster)  [unwired: 4 in]
                  n82 = case shown="Default" w537 {
                    selector: w537 -> [w547 w559 w573 w610 w618]
                    tunnel: w539 -> [w548 w552 w566 w608 w619]
                    tunnel: w543 -> [w549 w556 w563 w607 w614]
                    tunnel: w542 -> [w550 w555 w562 w606 w613]
                    tunnel: [w550 w555 w560 w606 w613] -> w541
                    tunnel: [w549 w556 w561 w607 w614] -> w540
                    tunnel: [w548 w553 w569 w608 w619] -> w538
                    tunnel: w536 -> [w546 w558 w570 w611 w617]
                    tunnel: [w547 w559 w572 w610 w618] -> w535
                    tunnel: [w546 w558 w571 w611 w617] -> w534
                    tunnel: [w545 w557 w575 w609 w616] -> w533
                    tunnel: w532 -> [w545 w557 w575 w609 w616]
                    tunnel: [w544 w554 w574 w612 w615] -> w531
                    tunnel: w530 -> [w544 w554 w574 w612 w615]
                    tunnel: w529 -> [_ _ _ _ _]
                    tunnel: [_ _ w565 _ _] -> w527
                    tunnel: w526 -> [_ _ w564 _ _]
                    frame Default {
                    }
                    frame "macro: initialize" {
                      n83 = call "Add State(s) to Queue__jkism.vi"("State(s) in Front (\"\")"="Macro: Initialize -><complete>" ("State(s) in Front (\"\")"), "State(s) in (\"\")"=w552) -> ("States Out"=w553:string)  [unwired: 13 in]
                    }
                    frame "macro: exit" {
                      w568 = "->[\\t\\s]*<[Ll][Oo]+[Pp]>[\\t\\s]*"  # -><loop>
                      # "#github 555 \nhttps://github.com/NEVSTOP-LAB/Communicable-State-Machine/issues/555\nwhen CSM enter Macro: Exit State, it will not process any states anymore."
                      # "if -><loop> is found, continous to parse next state"
                      # "#github 288 \nhttps://github.com/NEVSTOP-LAB/Communicable-State-Machine/issues/288\nWhen Macro: Exit is detected. CSM will stop LOOP firstly, then exit."
                      n84 = Match Pattern(string=w566, regular expression=w568) -> (offset past match=w567:i32)  [unwired: 1 in, 3 out]
                      n85 = Greater Or Equal To 0?(x=w567) -> (x >= 0?=w565:bool)
                      n86 = case shown="True" w565 {
                        tunnel: w573 -> [w578 _]
                        tunnel: [w578 _] -> w572
                        tunnel: [w577 _] -> w571
                        tunnel: w570 -> [w577 _]
                        tunnel: [w576 w591] -> w569
                        tunnel: w566 -> [w576 w581]
                        tunnel: w564 -> [_ w590]
                        frame False {
                        }
                        frame True {
                          w579 = "->[\\t\\s]*<[Ll][Oo]+[Pp]>[\\t\\s]*"  # -><loop>
                          w584 = "->[\\t\\s]*<[Ee][Nn][Dd]>[\\t\\s]*"  # -><end>
                          n87 = call "CSM - Break Down Multiple States String.vi"("States"=w581) -> ("Multiple States"=w582:string[])  [unwired: 10 in]
                          n88 = for {
                            tunnel: [w594] -> w583 mode=indexing if=w595
                            tunnel: w582 -> [w594] mode=indexing
                            tunnel: w579 -> [w592]
                            n89 = call "Remove Comments from Single-line.vi"("single-line text"=w594) -> ("single-line text without comments"=w593:string)  [unwired: 2 in]
                            n90 = Match Pattern(string=w593, regular expression=w592) -> (offset past match=w596:i32)  [unwired: 1 in, 3 out]
                            n91 = Less Than 0?(x=w596) -> (x < 0?=w595:bool)
                          }
                          n92 = call "CSM - Compact Multiple States.vi"("Multiple States"=w583) -> ("States"=w580:string)  [unwired: 9 in]
                          n93 = Match Pattern(string=w580, regular expression=w584) -> (before substring=w587:string, match substring=w588:string, after substring=w589:string, offset past match=w585:i32)  [unwired: 1 in]
                          n94 = Greater Or Equal To 0?(x=w585) -> (x >= 0?=w586:bool)
                          n95 = case shown="False" w586 {
                            tunnel: [w597 w603] -> w591
                            tunnel: w580 -> [w598 _]
                            tunnel: w587 -> [_ w605]
                            tunnel: w588 -> [_ w604]
                            tunnel: w589 -> [_ w600]
                            tunnel: w590 -> [w599 w601]
                            frame False {
                              n96 = call "Add State(s) to Queue__jkism.vi"("State(s) in Front (\"\")"=w599, "State(s) in (\"\")"=w598) -> ("States Out"=w597:string)  [unwired: 13 in]
                            }
                            frame True {
                              n97 = Concatenate Strings(w605, w604) -> (w602:string)
                              n98 = call "Add State(s) to Queue__jkism.vi"("State(s) in Front (\"\")"=w602, "State(s) in (\"\")"=w601, "State(s) at Back (\"\")"=w600) -> ("States Out"=w603:string)  [unwired: 12 in]
                            }
                          }
                        }
                      }
                      n99 = call "_CSMObj-Mark as Exiting.vi"("Error In"=w562, "CSMQ In"=w563) -> ("error out"=w560:errorcluster, "CSMQ Out"=w561:T3)  [unwired: 8 in]
                    }
                    frame "exit" {
                    }
                    frame "async response" {
                    }
                  }
                }
                frame Default {
                  # "Error, should not be here."
                }
              }
              n100 = call "CSM - Convert Error to Argument.vi"("Error"=w137) -> ("Argument"=w136:string)  [unwired: 4 in]
              n101 = Select(t="Critical Error", s=w137, f=w166) -> (s? t:f=w162:string)
              n102 = Select(t=w136, s=w137, f=w165) -> (s? t:f=w164:string)
              n103 = Empty String/Path?(string/path=w158) -> (empty?=w171:bool)
              n104 = Empty String/Path?(string/path=w162) -> (empty?=w172:bool)
              n105 = Not(x=w171) -> (.not. x?=w170:bool)
              n106 = And(x=w172, y=w170) -> (x .and. y?=w159:bool)
            }
          }
        }
        n107 = Empty String/Path?(string/path=w85) -> (empty?=w84:bool)
        n108 = And(x=w84, y=w86) -> (x .and. y?=w87:bool)
      }
    }
    frame Error {
      # "Goto Error Handler State >>"
      # "preserve remaining states >>"
      n109 = call "_CSMObj-Log Error if in a Remote Session.vi"("Error"=w630, "Error In"=w633, "CSMQ In"=w634) -> ("CSMQ Out"=w629:T3)  [unwired: 7 in, 1 out]
      n110 = call "CSM - Convert Error to Argument.vi"("Error"=w630) -> ("Argument"=w635:string)  [unwired: 4 in]
    }
  }
  n111 = feedback-in #1(w7) -> ()
  n112 = feedback-in #2(w3) -> ()
  n113 = in-place {
    in-place-border: w26 -> [w649]
    in-place-border: w11 -> [w651]
    in-place-border: w3 -> [w660]
    in-place-border: w2 -> [w640]
    n114 = in-place-match #3(w31) -> (w653:string)
    n115 = in-place-match #4(w27) -> (w646:string)
    n116 = in-place-match #5(w39) -> (w658:string)
    n117 = in-place-match #6(w38) -> (w657:string)
    n118 = in-place-match #7(w36) -> (w654:string)
    n119 = in-place-match #8(w37) -> (w655:string)
    n120 = in-place-match #9(w23) -> (w656:string)
    n121 = Unbundle By Name(w649) -> ("Valid"=w659:bool)
    n122 = case shown="True" w659 {
      tunnel: w649 -> [w808 w825]
      tunnel: w658 -> [w816 w824]
      tunnel: [w816 w824] -> w641
      tunnel: w657 -> [w815 w823]
      tunnel: [w815 w823] -> w645
      tunnel: [w814 w822] -> w643
      tunnel: w655 -> [w814 w822]
      tunnel: [w813 w820] -> w644
      tunnel: w654 -> [w813 w820]
      tunnel: w646 -> [w812 w819]
      tunnel: [w812 w819] -> w647
      tunnel: [w811 w826] -> w652
      tunnel: w653 -> [w811 w826]
      tunnel: [w810 w821] -> w642
      tunnel: w656 -> [w810 w821]
      tunnel: w651 -> [w809 w818]
      tunnel: [w809 w818] -> w650
      tunnel: [w808 w817] -> w648
      frame False {
      }
      frame True {
        n123 = call "GEvt-Generate State Change Log.vi"("CSM Global Log Event"=w825, "Current State"=w824, "Arguments"=w823, "Source Message.*State"=w822, "Source Message.*Arguments"=w821, "Source Module"=w820, "Name (\"\" to Use UUID)"=w819, "CSM:LogFilter.lvclass"=w818) -> ("CSM Global Log Event Out"=w817:T2)  [unwired: 10 in, 1 out]
      }
    }
    n124 = call "Auto Broadcast State.vi"("CSM Name"=w647, "Current State"=w641, "States Queue"=w652) -> ("Remaining States Queue"=w661:string)  [unwired: 6 in]
    n125 = case shown="\"Critical Error\", \"Exit\"" w641 {
      tunnel: [w664 w687] -> w663
      tunnel: [w665 w686] -> w662
      tunnel: w661 -> [w665 w683]
      tunnel: w660 -> [_ w679]
      tunnel: w650 -> [_ w670]
      tunnel: w648 -> [_ w668]
      tunnel: w647 -> [w664 w669]
      tunnel: w640 -> [_ w677]
      frame Default {
      }
      frame "Critical Error", "Exit" {
        # "#github\nmove it here to release registration when\ncritical error occured."
        # "#github \nThis is used to process:\n1. Sync/Async message of \"Macro: Exit\",\"Exit\",\"Critical Error\"\n2. State registration of \"Macro: Exit\",\"Exit\",\"Critical Error\""
        n126 = call "_CSMObj-Unregister Internal Registry Rules.vi"("CSM:LogFilter.lvclass"=w670, "Name (\"\" to Use UUID)"=w669, "CSM Global Log Event"=w668, "CSMQ In"=w677) -> ("error out"=w672:errorcluster, "CSMQ Out"=w674:T3)  [unwired: 6 in]
        n127 = call "_CSMObj-Lock State.vi"("Error In"=w672, "CSMQ In"=w674) -> ("error out"=w673:errorcluster, "CSMQ Out"=w671:T3, "Error"=w676:errorcluster)  [unwired: 5 in, 1 out]
        n128 = call "_CSMObj-Unlock.vi"("Error In"=w673, "CSMQ In"=w671) -> ("error out"=w667:errorcluster, "CSMQ Out"=w675:T3)  [unwired: 8 in]
        n129 = call "Parse Action State After Exit.vi"("States"=w683) -> ("Need to Process"=w678:string, "Remaining States"=w684:string)  [unwired: 9 in]
        n130 = call "_CSMOFGV Release.vi"("Error In"=w667, "CSMQ"=w675) -> ("error out"=w666:errorcluster)  [unwired: 9 in]
        n131 = case shown="Default" w678 {
          selector: w678 -> [_ w693]
          tunnel: w669 -> [w690 w700]
          tunnel: w668 -> [w689 w699]
          tunnel: [w690 w698] -> w680
          tunnel: [w689 w697] -> w681
          tunnel: w670 -> [w688 w696]
          tunnel: [w688 w695] -> w682
          tunnel: w679 -> [_ w694]
          tunnel: w676 -> [_ w691]
          tunnel: w666 -> [_ _]
          frame "" {
          }
          frame Default {
            n132 = call "CSM - Break Down Multiple States String.vi"("States"=w693) -> ("Multiple States"=w692:string[])  [unwired: 10 in]
            n133 = for "While current line is a comment and there are more lines to process" {
              shift-right: [w705] -> w698
              shift-left: w700 -> [w717]
              shift-right: [w703] -> w697
              shift-left: w699 -> [w716]
              shift-right: [w704] -> w695
              shift-left: w696 -> [w706]
              tunnel: w694 -> [w707]
              tunnel: w692 -> [w702] mode=indexing
              tunnel: w691 -> [w701]
              # "source/target"
              # "Pre-Args"
              # "Pre-State"
              # "name"
              # "remaining lines"
              # "args"
              # "state"
              n134 = call "Remove Comments from Single-line.vi"("single-line text"=w702) -> ("single-line text without comments"=w715:string)  [unwired: 2 in]
              n135 = call "Split Single-line Message.vi"("single-line text"=w715) -> ("operator"=w712:string, "state"=w713:string, "args"=w714:string, "source/target"=w711:string)  [unwired: 6 in]
              n136 = call "Split Single-line Reason Parts.vi"("Single-line -& Reason"=w711) -> ("CSM Name"=w710:string, "`State"=w709:string, "`Arguments"=w708:string)  [unwired: 12 in]
              n137 = case shown="\"-&\"" w712 {
                selector: w712 -> [w724 _ _]
                tunnel: w713 -> [w727 w760 _]
                tunnel: w714 -> [w726 w761 _]
                tunnel: w717 -> [w725 w759 w798]
                tunnel: w710 -> [w728 w758 _]
                tunnel: w716 -> [w723 w750 w799]
                tunnel: [w722 w749 w799] -> w703
                tunnel: [w721 w753 w798] -> w705
                tunnel: w709 -> [_ w757 _]
                tunnel: w708 -> [_ w756 _]
                tunnel: w706 -> [w720 w752 w797]
                tunnel: w707 -> [w719 _ _]
                tunnel: [w718 w751 w797] -> w704
                tunnel: w701 -> [_ w755 _]
                frame "->", "->|" {
                  # "Async Call and post message to other loop"
                  n138 = case shown="\"<state>\"" w728 {
                    selector: w728 -> [_ w734]
                    tunnel: w727 -> [_ w740]
                    tunnel: w726 -> [_ w738]
                    tunnel: w725 -> [w730 w739]
                    tunnel: w724 -> [_ _]
                    tunnel: [w731 w741] -> w722
                    tunnel: w723 -> [w731 w742]
                    tunnel: [w730 w739] -> w721
                    tunnel: w720 -> [w729 w733]
                    tunnel: w719 -> [_ w735]
                    tunnel: [w729 w733] -> w718
                    frame Default {
                    }
                    frame "<state>" {
                      n139 = call "Replace LastResp Token.vi"("LastResp"="" ("Response Before \"Error Handler\""), "Argument"=w738) -> ("Argument Out"=w736:string)  [unwired: 5 in]
                      n140 = call "GEvt-Generate Status Log.vi"("CSM Global Log Event"=w742, "Current State"=w740, "Arguments"=w736, "Source Module"=w734, "Name (\"\" to Use UUID)"=w739, "CSM:LogFilter.lvclass"=w733) -> ("CSM Global Log Event Out"=w741:T2)  [unwired: 12 in, 1 out]
                      n141 = call "Cache-StatusChangeEventRef.vi"("Name (\"\" to Use UUID) In"=w739) -> ("Status Event"=w743:refnum<user-event>)  [unwired: 8 in, 2 out]
                      n142 = Bundle(cluster=T13 {"ModuleName"="", "Status"="", "Arguments"=""} ("event data"), "ModuleName"=w739, "Status"=w740, "Arguments"=w736) -> (w744:T13)
                      n143 = Not A Number/Path/Refnum?(number/path/refnum=w743) -> (NaN/Path/Refnum?=w746:bool)
                      n144 = case shown="False" w746 {
                        tunnel: w743 -> [w748 _]
                        tunnel: w744 -> [w747 _]
                        frame False {
                          n145 = Generate User Event(user event=w748, event data cluster=w747) -> ()  [unwired: 2 in, 2 out]
                        }
                        frame True {
                        }
                      }
                      n146 = call "CSMP-Broadcast.vi"("State"=w740, "Args"=w736, "Source/target"=w734, "Response For Message.’Error"=w735, "Module Name"=w739, "Msg Type"=_CSM_MSG_TYPE."Broadcast(-><state>)") -> ()  [unwired: 8 in, 6 out]
                    }
                  }
                }
                frame "-&" {
                  # "Synchonized Call send msg and wait response"
                  n147 = case shown="\"PostPostMsg\"" w760 {
                    selector: w760 -> [_ w781 w796]
                    tunnel: w758 -> [_ w765 w783]
                    tunnel: w761 -> [_ w780 w795]
                    tunnel: "" ("Response Before \"Error Handler\"") -> [_ w782 w793]
                    tunnel: w759 -> [w764 w775 w786]
                    tunnel: w757 -> [_ w774 w785]
                    tunnel: w756 -> [_ w773 w784]
                    tunnel: w755 -> [_ w779 w794]
                    tunnel: [w764 w775 w786] -> w753
                    tunnel: w752 -> [w763 w770 w787]
                    tunnel: [w763 w770 w787] -> w751
                    tunnel: w750 -> [w762 w769 w789]
                    tunnel: [w762 w768 w788] -> w749
                    frame Default {
                    }
                    frame "PostPostMsg" {
                      n148 = call "CSMP-PostPostMsg.vi"("State"=w781, "Args"=w780, "Source/target"=w765, "Pre-State In"=w774, "Pre-Args In"=w773, "Session Error"=w779, "Module Name"=w775, "Response Arguments"=w782) -> ("Pre-State Out"=w767:string, "Pre-Args Out"=w766:string)  [unwired: 6 in, 4 out]
                      n149 = Empty String/Path?(string/path=w765) -> (empty?=w772:bool)
                      n150 = Bundle By Name(cluster=T12 {"Name (\"\" to Use UUID)"="", "Current State"="", "Arguments"="", "Source Message"={"‘State"="", "’Arguments"="", "’Error"={"status"=FALSE, "code"=0, "source"=""}}, "Source Module"="", "Complete(T)/Start(F)"=FALSE, "LogType"=enum."State Change", "Time Stamp"=timestamp(0 s since 1904-01-01)} ("Event Data"), "Name (\"\" to Use UUID)"=w775, "Current State"=w767, "Arguments"=w766, "Source Module"=w765, "LogType"=_CSM_GlobalLog_MSG_TYPE."Async Message") -> (w776:T12)
                      n151 = Not(x=w772) -> (.not. x?=w771:bool)
                      n152 = call "GEvt-Generate Complete Log.vi"("CSM Global Log Event"=w769, "Event Data"=w776, "Enable?"=w771, "CSM:LogFilter.lvclass"=w770) -> ("CSM Global Log Event Out"=w768:T2)  [unwired: 15 in]
                    }
                    frame "PostSendMsg" {
                      n153 = call "CSMP-PostSendMsg.vi"("State"=w796, "Args"=w795, "Source/target"=w783, "Session Error"=w794, "Module Name"=w786, "Response Arguments"=w793) -> ()  [unwired: 10 in, 4 out]
                      n154 = Bundle By Name(cluster=T12 {"Name (\"\" to Use UUID)"="", "Current State"="", "Arguments"="", "Source Message"={"‘State"="", "’Arguments"="", "’Error"={"status"=FALSE, "code"=0, "source"=""}}, "Source Module"="", "Complete(T)/Start(F)"=FALSE, "LogType"=enum."State Change", "Time Stamp"=timestamp(0 s since 1904-01-01)} ("Event Data"), "Name (\"\" to Use UUID)"=w786, "Current State"=w785, "Arguments"=w784, "Source Module"=w783, "LogType"=_CSM_GlobalLog_MSG_TYPE."Sync Message") -> (w790:T12)
                      n155 = call "GEvt-Generate Complete Log.vi"("CSM Global Log Event"=w789, "Event Data"=w790, "CSM:LogFilter.lvclass"=w787) -> ("CSM Global Log Event Out"=w788:T2)  [unwired: 16 in]
                    }
                  }
                }
                frame Default {
                  # "Error, should not be here."
                }
              }
            }
          }
        }
        n156 = Unbundle By Name(w681) -> ("Valid"=w685:bool)
        n157 = case shown="True" w685 {
          tunnel: w681 -> [_ w803]
          tunnel: w680 -> [w801 w805]
          tunnel: [w801 w805] -> w687
          tunnel: [w800 w807] -> w686
          tunnel: w684 -> [w800 w807]
          tunnel: w682 -> [_ w804]
          frame False {
          }
          frame True {
            w802 = TRUE ("Enable?")
            n158 = call "GEvt-Generate Remaining States Log.vi"("CSM Global Log Event"=w803, "Remaining States"=w807, "Name (\"\" to Use UUID)"=w805, "Enable?"=w802, "CSM:LogFilter.lvclass"=w804) -> ("CSM Global Log Event Out"=w806:T2)  [unwired: 13 in, 1 out]
            n159 = call "GEvt-Generate Module Destroyed Log.vi"("CSM Global Log Event"=w806, "Name (\"\" to Use UUID)"=w805, "Enable?"=w802, "CSM:LogFilter.lvclass"=w804) -> ()  [unwired: 14 in, 2 out]
          }
        }
      }
    }
    n160 = in-place-match #3(w662) -> (→"Remaining States":string)
    n161 = in-place-match #4(w663) -> (→"Name Used":string)
    n162 = in-place-match #5(w641) -> (→"Current State":string)
    n163 = in-place-match #6(w645) -> (→"Arguments":string)
    n164 = in-place-match #7(w644) -> (→"Source CSM":string)
    n165 = in-place-match #8(w643) -> (w25:string)
    n166 = in-place-match #9(w642) -> (w22:string)
  }
  n167 = Bundle By Name(cluster=T1 {"‘State"="", "’Arguments"="", "’Error"={"status"=FALSE, "code"=0, "source"=""}} (">> Response Source Message >>"), "‘State"=w25, "’Arguments"=w22, "’Error"=w20) -> (→"Additional Information":T1)
